vi "GOOP_GetClassProvider.vi"(1 "New Item Parent/Object":variant, 3 "CreateClass":bool, 5 "error in (no error)":errorcluster, 6 "ProviderClassType":T1) -> (15 "ProjectItem":refnum<vi>, 16 "LVClass.Open":refnum<vi>, 19 "error out":errorcluster)   [LabVIEW 2020]
uses:
  GOOP_ClassProviderClassType.ctl
  <resource>/Framework/Providers/API/mxLvNIIM.ctl
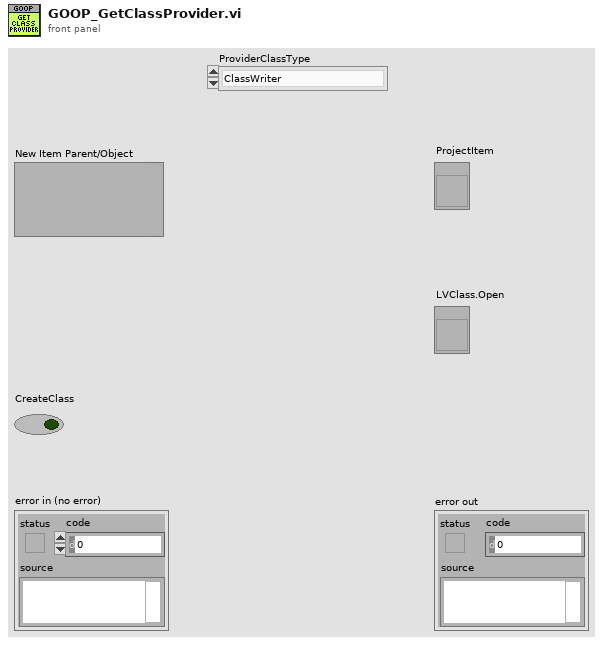
[diagram p1: front panel]
types:
  T1 = typedef "GOOP_ClassProviderClassType.ctl" = enum16{"ClassWriter", "ClassReader"}
  T2 = typedef "mxLvNIIM.ctl" = cluster{"Item URL":string, "Item ID":string, "Item Index":i32, "Specific Type":string}
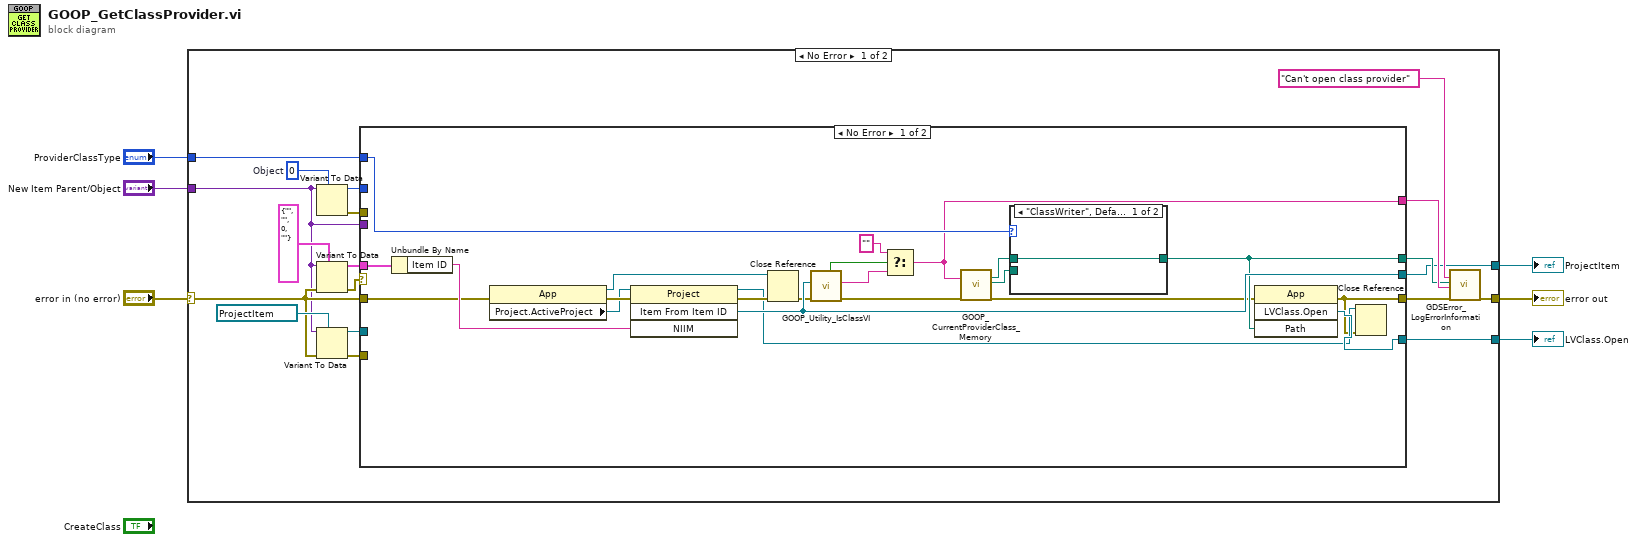
[diagram p0: block diagram]
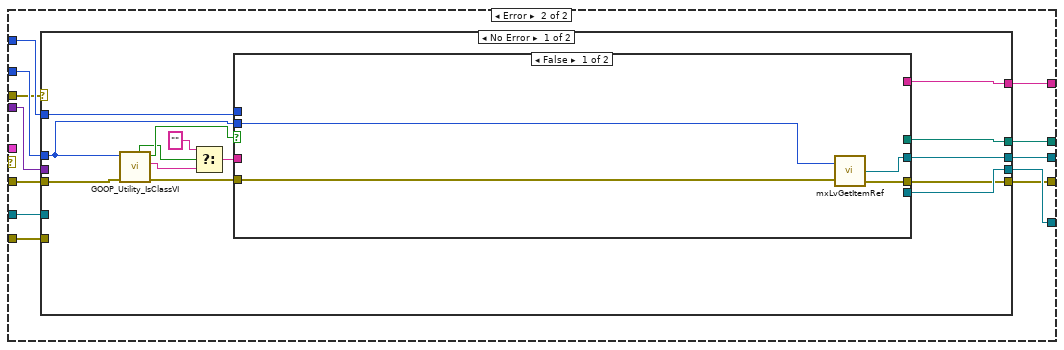
[diagram p3: hidden frame]
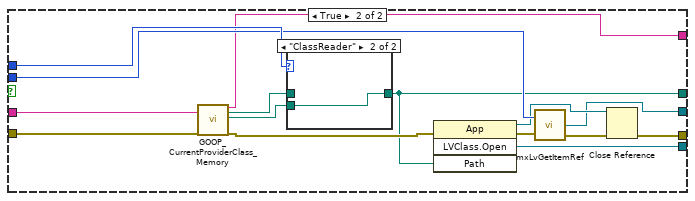
[diagram p4: hidden frame]
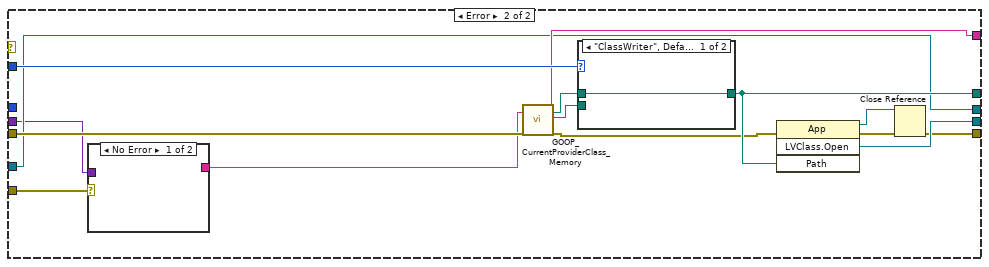
[diagram p6: hidden frame]
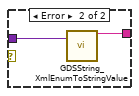
[diagram p7: hidden frame]
diagram:
  n1 = case shown="No Error" "error in (no error)" {
    selector: "error in (no error)" -> [w10 w116]
    tunnel: [w15 _] -> w2
    tunnel: [w13 _] -> w3
    tunnel: [w19 w116] -> w4
    tunnel: "New Item Parent/Object" -> [w7 _]
    tunnel: "ProviderClassType" -> [w20 _]
    frame No Error {
      w23 = u64 0  # Object
      n2 = Variant To Data(type=w23, Variant=w7) -> (data=w22:u64, error out=w12:errorcluster)  [unwired: 1 in]
      n3 = Variant To Data(error in=w10, type=T2 {"Item URL"="", "Item ID"="", "Item Index"=0, "Specific Type"=""} ("New Item Parent"), Variant=w7) -> (data=w24:T2, error out=w21:errorcluster)
      n4 = Variant To Data(error in=w10, type=refnum<vi> refnum ("My Computer"), Variant=w7) -> (data=w8:refnum<vi>, error out=w9:errorcluster)
      n5 = case shown="No Error" w21 {
        tunnel: [w47 w57] -> w15
        tunnel: [w39 w58] -> w13
        tunnel: w10 -> [w30 w61]
        tunnel: [w32 w56] -> w18
        tunnel: w24 -> [w44 _]
        tunnel: w22 -> [_ w59]
        tunnel: w20 -> [w36 w60]
        tunnel: [w26 w55] -> w17
        tunnel: [w37 w54] -> w14
        tunnel: w12 -> [_ w53]
        tunnel: w9 -> [_ w52]
        tunnel: w8 -> [_ w51]
        tunnel: w7 -> [_ w50]
        frame No Error {
          n6 = Unbundle By Name(w44) -> ("Item ID"=w42:string)
          n7 = property class="App"(error in=w30) -> (reference out=w45:refnum<vi>, error out=w43:errorcluster, "Project.ActiveProject"=w35:refnum<vi>)  [unwired: 1 in]
          n8 = invoke class="Project" method="Item From Item ID"(reference=w35, error in=w43, "NIIM"=w42) -> (reference out=w33:refnum<vi>, error out=w46:errorcluster, "GetItemFromNIIM"=w39:refnum<vi>)  [unwired: 1 in, 1 out]
          n9 = Close Reference(reference=w45, error in (no error)=w46) -> (error out=w34:errorcluster)
          n10 = call "GOOP_Utility_IsClassVI.vi"("error in (no error)"=w34, "ProjectItem"=w39) -> ("error out"=w38:errorcluster, "ClassProvider"=w27:string, "Is Interface?"=w28:bool)  [unwired: 4 in, 3 out]
          n11 = Select(t="", s=w28, f=w27) -> (s? t:f=w26:string)
          n12 = call "GOOP_CurrentProviderClass_Memory.vi"("GetThisClassProvidersPaths(Returns the default providor if not wired)"=w26, "error in (no error)"=w38) -> ("ClassProviderClassWriterPath"=w40:path, "ClassProviderClassReaderPath"=w41:path, "error out"=w31:errorcluster)  [unwired: 11 in, 4 out]
          n13 = case shown="\"ClassWriter\", Default" w36 {
            tunnel: w41 -> [_ w49]
            tunnel: [w48 w49] -> w37
            tunnel: w40 -> [w48 _]
            frame "ClassWriter", Default {
            }
            frame "ClassReader" {
            }
          }
          n14 = invoke class="App" method="LVClass.Open"(error in=w31, "Path"=w37) -> (error out=w32:errorcluster, "LVClass.Open"=w47:refnum<vi>)  [unwired: 2 in, 2 out]
          n15 = Close Reference(reference=w33, error in (no error)=w32) -> ()  [unwired: 1 out]
        }
        frame Error {
          n16 = case shown="No Error" w53 {
            tunnel: w61 -> [w75 w107]
            tunnel: w60 -> [w73 w111]
            tunnel: w59 -> [w72 _]
            tunnel: [w71 w100] -> w58
            tunnel: [w70 w110] -> w57
            tunnel: [w69 w109] -> w56
            tunnel: [w66 w106] -> w55
            tunnel: [w67 w108] -> w54
            tunnel: w52 -> [_ w97]
            tunnel: w51 -> [_ w100]
            tunnel: w50 -> [_ w99]
            frame No Error {
              n17 = call "GOOP_Utility_IsClassVI.vi"("error in (no error)"=w75, "Object"=w72) -> ("error out"=w74:errorcluster, "ClassProvider"=w64:string, "Is Class VI?"=w68:bool, "Is Interface?"=w65:bool)  [unwired: 4 in, 2 out]
              n18 = Select(t="", s=w65, f=w64) -> (s? t:f=w63:string)
              n19 = case shown="False" w68 {
                tunnel: w74 -> [w79 w92]
                tunnel: w63 -> [_ w91]
                tunnel: w73 -> [_ w89]
                tunnel: w72 -> [w77 w87]
                tunnel: [w76 w82] -> w71
                tunnel: [_ w83] -> w70
                tunnel: [w78 w84] -> w69
                tunnel: [_ w81] -> w67
                tunnel: [_ w80] -> w66
                frame False {
                  n20 = call <resource>:"mxLvGetItemRef.vi"("Item"=w77, "error in"=w79) -> ("Item Refnum"=w76:refnum<vi>, "error out"=w78:errorcluster)  [unwired: 1 out]
                }
                frame True {
                  n21 = call "GOOP_CurrentProviderClass_Memory.vi"("GetThisClassProvidersPaths(Returns the default providor if not wired)"=w91, "error in (no error)"=w92) -> ("ClassProviderName"=w80:string, "ClassProviderClassWriterPath"=w93:path, "ClassProviderClassReaderPath"=w94:path, "error out"=w90:errorcluster)  [unwired: 11 in, 3 out]
                  n22 = case shown="\"ClassReader\"" w89 {
                    tunnel: w94 -> [_ w96]
                    tunnel: [w95 w96] -> w81
                    tunnel: w93 -> [w95 _]
                    frame "ClassWriter", Default {
                    }
                    frame "ClassReader" {
                    }
                  }
                  n23 = invoke class="App" method="LVClass.Open"(error in=w90, "Path"=w81) -> (reference out=w85:refnum<vi>, error out=w88:errorcluster, "LVClass.Open"=w83:refnum<vi>)  [unwired: 2 in, 1 out]
                  n24 = call <resource>:"mxLvGetItemRef.vi"("Item"=w87, "error in"=w88) -> ("Item Refnum"=w82:refnum<vi>, "error out"=w86:errorcluster)  [unwired: 1 out]
                  n25 = Close Reference(reference=w85, error in (no error)=w86) -> (error out=w84:errorcluster)
                }
              }
            }
            frame Error {
              n26 = case shown="No Error" w97 {
                tunnel: w99 -> [_ w113]
                tunnel: [_ w112] -> w98
                frame No Error {
                }
                frame Error {
                  n27 = call "GDSString_XmlEnumToStringValue.vi"("EnumVariantIn(used if String is Empty)"=w113) -> ("EnumValueOut(string)"=w112:string)  [unwired: 15 in, 3 out]
                }
              }
              n28 = call "GOOP_CurrentProviderClass_Memory.vi"("GetThisClassProvidersPaths(Returns the default providor if not wired)"=w98, "error in (no error)"=w107) -> ("ClassProviderName"=w106:string, "ClassProviderClassWriterPath"=w104:path, "ClassProviderClassReaderPath"=w105:path, "error out"=w103:errorcluster)  [unwired: 11 in, 3 out]
              n29 = case shown="\"ClassWriter\", Default" w111 {
                tunnel: w105 -> [_ w115]
                tunnel: [w114 w115] -> w108
                tunnel: w104 -> [w114 _]
                frame "ClassWriter", Default {
                }
                frame "ClassReader" {
                }
              }
              n30 = invoke class="App" method="LVClass.Open"(error in=w103, "Path"=w108) -> (reference out=w102:refnum<vi>, error out=w101:errorcluster, "LVClass.Open"=w110:refnum<vi>)  [unwired: 2 in, 1 out]
              n31 = Close Reference(reference=w102, error in (no error)=w101) -> (error out=w109:errorcluster)
            }
          }
        }
      }
      n32 = call "GDSError_LogErrorInformation.vi"("State"="Can't open class provider", "LocalVariableData"=w14, "ExtraErrorInfo"=w17, "error in (no error)"=w18) -> ("error out"=w19:errorcluster)  [unwired: 15 in]
    }
    frame Error {
    }
  }
  "error out" <- w4
  "LVClass.Open" <- w2
  "ProjectItem" <- w3
